vi "Setup Auto.vi"() -> (3 "Auto Data":T1)   [LabVIEW 2027]
uses:
  Drive/Implementation/Auto Data.ctl
  swerve-template/Type Definitions/Data/Robot Velocities.ctl
  Drive Conditions.ctl
  239c1ceb-589e-4f7c-8125-dfea88b83b5c.vi
  <vilib>/Rock Robotics/Network Tables/NT Read String.vi
  <vilib>/Rock Robotics/Network Tables/NT Read String Array.vi
  <vilib>/Utility/file.llb/Read Delimited Spreadsheet (string).vi
  Robot Global Data.vi
  <vilib>/Rock Robotics/Network Tables/NT Read Boolean.vi
  <vilib>/MRC/MrcLib.lvlib
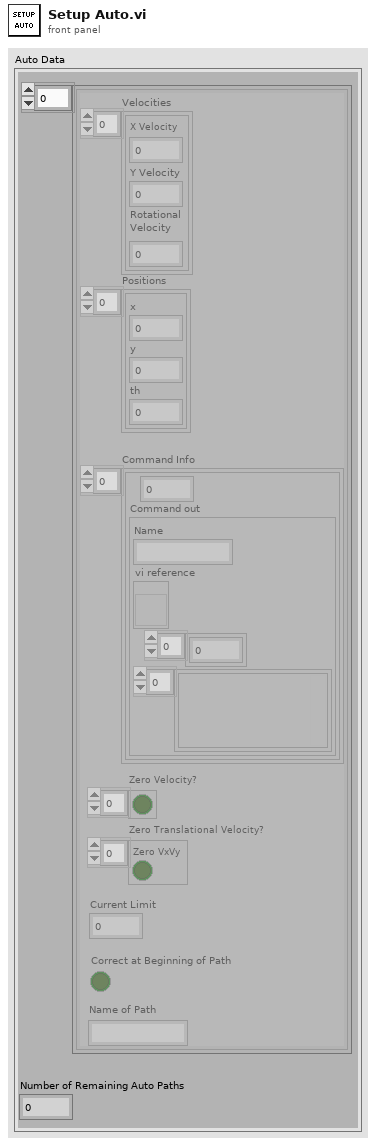
[diagram p1: front panel]
types:
  T1 = typedef "Auto Data.ctl" = cluster{"Auto Data":cluster{"Velocities":T2[], "Positions":cluster{"x":dbl, "y":dbl, "th":dbl}[], "Command Info":cluster{dbl, "Command out":cluster{"Name":string, "vi reference":refnum<vi>, i32[], variant[]}}[], "Zero Velocity?":bool[], "Zero Translational Velocity?":bool[], "Current Limit":dbl, "Correct at Beginning of Path":bool, "Name of Path":string}[], "Number of Remaining Auto Paths":dbl}
  T2 = typedef "Robot Velocities.ctl" = cluster{"X Velocity":dbl, "Y Velocity":dbl, "Rotational \nVelocity":dbl}
  T3 = typedef "Drive Conditions.ctl" = cluster{"Field Centric":bool, "Reset PIDs":bool}
  T4 = typedef "Single Cmd Info.ctl" = cluster{"Name":string, "CPTM.DataType":variant, "All Control Values Variant":cluster{"Name":string, "Variant Data":variant}[], "icon full":T5, "icon scaled":T5, "Path":path, "Subsystem Color":u32}
  T5 = typedef "imagedata.ctl" = cluster{"image type":i32, "image depth":i32, "image":u8[], "mask":u8[], "colors":u32[], "Rectangle":cluster{"left":i16, "top":i16, "right":i16, "bottom":i16}}
  T6 = cluster{"Name":string, "vi reference":refnum<vi>, i32[], variant[]}
  T7 = cluster{"Time (s)":dbl, "Command out":cluster{"Name":string, "vi reference":refnum<vi>, i32[], variant[]}}
  T8 = cluster{"Time (s)":dbl, "Command out":cluster{"Name":string, "vi reference":refnum<vi>, i32[], variant[]}}[]
  T9 = cluster{"Velocities":T2[], "Positions":cluster{"x":dbl, "y":dbl, "th":dbl}[], cluster{"Time (s)":dbl, "Command out":cluster{"Name":string, "vi reference":refnum<vi>, i32[], variant[]}}[], "Zero Velocity?":bool[], "Zero Translational Velocity?":bool[], "Current Limit":dbl, "Correct at Beginning \nof Path":bool, "String":string}
  T10 = cluster{cluster{"Velocities":T2[], "Positions":cluster{"x":dbl, "y":dbl, "th":dbl}[], cluster{"Time (s)":dbl, "Command out":cluster{"Name":string, "vi reference":refnum<vi>, i32[], variant[]}}[], "Zero Velocity?":bool[], "Zero Translational Velocity?":bool[], "Current Limit":dbl, "Correct at Beginning \nof Path":bool, "String":string}[], i32}
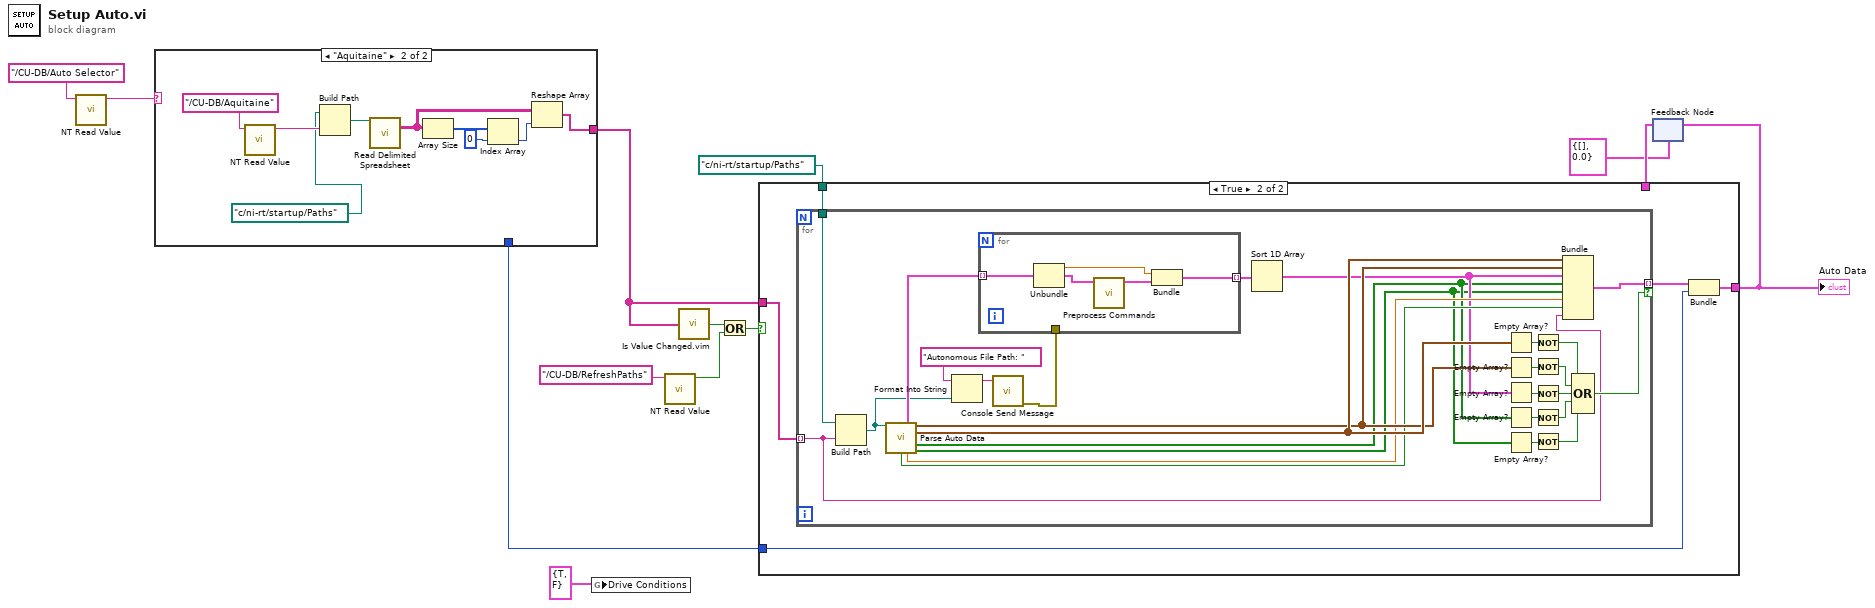
[diagram p0: block diagram]
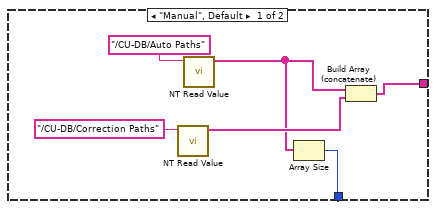
[diagram p3: hidden frame]
diagram:
  n1 = call-poly <vilib>:"NT Read Value.vi"("name"="/CU-DB/Auto Selector") -> ("value"=w13:string)  [unwired: 8 in, 2 out]
  n2 = case shown="\"Aquitaine\"" w13 {
    tunnel: [w16 w21] -> w10
    tunnel: [w14 _] -> w4
    frame "Manual", Default {
      n3 = call-poly <vilib>:"NT Read Value.vi"("name"="/CU-DB/Correction Paths") -> ("value"=w17:string[])  [unwired: 8 in, 2 out]
      n4 = call-poly <vilib>:"NT Read Value.vi"("name"="/CU-DB/Auto Paths") -> ("value"=w15:string[])  [unwired: 8 in, 2 out]
      n5 = Array Size(array=w15) -> (size(s)=w14:i32)
      n6 = Build Array (concatenate)(w15, w17) -> (w16:string[])
    }
    frame "Aquitaine" {
      n7 = call-poly <vilib>:"NT Read Value.vi"("name"="/CU-DB/Aquitaine") -> ("value"=w27:string)  [unwired: 8 in, 2 out]
      n8 = Build Path(base path=path "c:/ni-rt/startup/Paths" ("appended path"), name or relative path=w27) -> (appended path=w26:path)
      n9 = call-poly <vilib>:"Read Delimited Spreadsheet.vi"("file path (dialog if empty)"=w26) -> ("all rows"=w22:string[][])  [unwired: 9 in, 5 out]
      n10 = Array Size(array=w22) -> (size(s)=w25:i32[])
      n11 = Index Array(array=w25, index=0) -> (element=w23:i32)
      n12 = Reshape Array(w22, w23) -> (w21:string[])
    }
  }
  n13 = global write "Robot Global Data.vi" "Drive Conditions"(T3 {"Field Centric"=TRUE, "Reset PIDs"=FALSE} ("Drive Conditions")) -> ()
  n14 = call-poly <vilib>:"NT Read Value.vi"("name"="/CU-DB/RefreshPaths" ("Name")) -> ("value"=w6:bool)  [unwired: 8 in, 2 out]
  n15 = call "Is Value Changed.vim"("value"=w10) -> ("changed or first call?"=w7:bool)
  n16 = Or(x=w7, y=w6) -> (x .or. y?=w5:bool)
  n17 = feedback #1(T1 {"Auto Data"=[], "Number of Remaining Auto Paths"=0.0} ("Cluster")) -> (w9:T1)
  n18 = case shown="True" w5 {
    tunnel: [w29 w31] -> w2
    tunnel: w10 -> [_ w34]
    tunnel: w9 -> [w29 _]
    tunnel: w4 -> [_ w32]
    tunnel: path "c:/ni-rt/startup/Paths" ("appended path") -> [_ w30]
    frame False {
    }
    frame True {
      n19 = for {
        tunnel: w34 -> [w38] mode=indexing
        tunnel: [w53] -> w33 mode=indexing if=w39
        tunnel: w30 -> [w35]
        n20 = Build Path(base path=w35, name or relative path=w38) -> (appended path=w60:path)
        n21 = call "Parse Auto Data.vi"("path"=w60) -> ("Commands out"=w61:cluster{"Time (s)":dbl, T4, bool}[], "Positions"=w57:cluster{"x":dbl, "y":dbl, "th":dbl}[], "Velocities"=w58:T2[], "Zero Velocity?"=w51:bool[], "Correct at Beginning \nof Path"=w54:bool, "Current Limit"=w55:dbl, "Zero Translational Velocity?"=w50:bool[])  [unwired: 6 in, 2 out]
        n22 = Format Into String(initial string="Autonomous File Path: ", w60) -> (resulting string=w37:string)  [unwired: 2 in, 1 out]
        n23 = call <vilib>:"Console Send Message.vi"("Message"=w37) -> ("error out"=w36:errorcluster)  [unwired: 14 in]
        n24 = for {
          tunnel: w61 -> [w65] mode=indexing
          tunnel: [w62] -> w56 mode=indexing
          tunnel: w36 -> [_]
          n25 = Unbundle(w65) -> ("Time (s)"=w66:dbl, w64:T4)  [unwired: 1 out]
          n26 = call "Preprocess Commands.vi"("Command In"=w64) -> ("Command out"=w63:T6)  [unwired: 10 in]
          n27 = Bundle("Time (s)"=w66, "Command out"=w63) -> (w62:T7)  [unwired: 1 in]
        }
        n28 = Sort 1D Array(array=w56) -> (sorted array=w52:T8)
        n29 = Empty Array?(array=w58) -> (empty?=w49:bool)
        n30 = Empty Array?(array=w57) -> (empty?=w48:bool)
        n31 = Empty Array?(array=w52) -> (empty?=w47:bool)
        n32 = Empty Array?(array=w51) -> (empty?=w46:bool)
        n33 = Empty Array?(array=w50) -> (empty?=w45:bool)
        n34 = Not(x=w49) -> (.not. x?=w42:bool)
        n35 = Not(x=w48) -> (.not. x?=w43:bool)
        n36 = Not(x=w47) -> (.not. x?=w44:bool)
        n37 = Not(x=w46) -> (.not. x?=w41:bool)
        n38 = Not(x=w45) -> (.not. x?=w40:bool)
        n39 = Bundle("Velocities"=w58, "Positions"=w57, w52, "Zero Velocity?"=w51, "Zero Translational Velocity?"=w50, "Current Limit"=w55, "Correct at Beginning \nof Path"=w54, "String"=w38) -> (w53:T9)  [unwired: 1 in]
        n40 = Compound Arithmetic op=OR(w42, w43, w44, w41, w40) -> (w39:bool)
      }
      n41 = Bundle(w33, w32) -> (w31:T10)  [unwired: 1 in]
    }
  }
  "Auto Data" <- w2
  n42 = feedback-in #1(w2) -> ()
